vi "Empty Channel Settings.vi"() -> (0 "Channel Settings":T1={"Name"="", "Terminal Information"={"IO Device"=enum."none", "Channel"=0, "Sensor Type"=enum."Voltage"}, "Calibration Information"={"Excitation Voltage"=0.0, "Calibration Factor"=0.0, "Zero Value"=0.0, "Calibration Formula"="(x-x0) / (Ve * CF)", "Units"=""}})   [LabVIEW 2021, in "Acquisition.lvlib"]
doc: "(inline VI) Return an empty Channel Settings value. Use in-place of a block diagram constant.\n\nA cluster that holds the settings for a sensor channel."
uses:
  Acquisition.lvlib
  Channel Settings.ctl
  IO Device.ctl
  Sensor Type.ctl
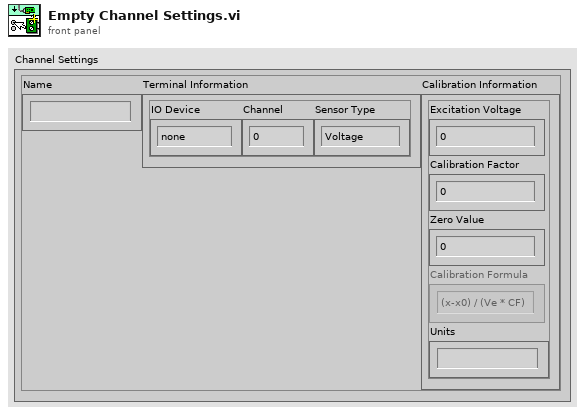
[diagram p1: front panel]
types:
  T1 = typedef "Acquisition.lvlib/Channel Settings.ctl" = cluster{"Name":string, "Terminal Information":cluster{"IO Device":T2, "Channel":i32, "Sensor Type":T3}, "Calibration Information":cluster{"Excitation Voltage":dbl, "Calibration Factor":dbl, "Zero Value":dbl, "Calibration Formula":string, "Units":string}}
  T2 = typedef "Acquisition.lvlib/IO Device.ctl" = enum16{"none", "9219", "9401"}
  T3 = typedef "Acquisition.lvlib/Sensor Type.ctl" = enum16{"Voltage", "Load", "Pressure", "Encoder"}
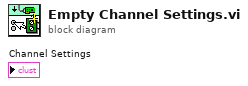
[diagram p0: block diagram]
diagram:
